vi "Create Group Commands.vi"(7 "VolatusAPI":refnum<class "VolatusAPI.lvclass">, 8 "error in (no error)":errorcluster, 9 "Group Name":string, 10 "Local Node":string, 11 "Cluster":refnum<class "Cluster Config.lvclass">) -> (0 "error out":errorcluster, 2 "Commands":T1)   [LabVIEW 2025, in "VolatusControl.lvlib" / "EStop Module.lvclass"]
uses:
  EStop Module.lvclass
  EStop Module.lvclass/EStop Module.ctl
  VolatusConfig/Channel/Channel Config.lvclass
  C:/dev/volatus/mts-volatus-super/libs/lv-volatus/VolatusConfig/VolatusConfigElement/VolatusConfigElement.lvclass
  C:/dev/volatus/mts-volatus-super/libs/lv-volatus/VolatusConfig/Channel/Channel Config.lvclass
  VolatusConfig/Node/Node Config.lvclass
  C:/dev/volatus/mts-volatus-super/libs/lv-volatus/VolatusConfig/Node/Node Config.lvclass
  VolatusConfig/Cluster/Cluster Config.lvclass
  VolatusConfig/Group/Group Config.lvclass
  VolatusConfig/VolatusConfigElement/VolatusConfigElement.lvclass
  messages/CmdDigital/Data.ctl
  messages/CmdDigital/CmdDigital.lvlib
  Volatus/VolatusAPI/VolatusAPI.lvclass
  lv-cdm/CDM-Config/Config Element/Config Element.lvclass
  Digital Group.ctl
  messages/CmdDigitalMultiple/Data.ctl
  messages/CmdDigitalMultiple/CmdDigitalMultiple.lvlib
  Volatus/MessageQ/MessageQ.lvclass
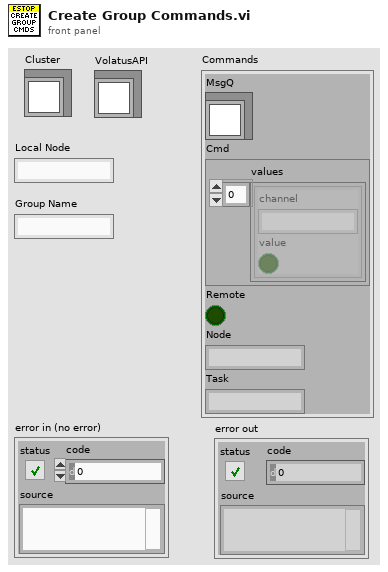
[diagram p1: front panel]
types:
  T1 = typedef "VolatusControl.lvlib/EStop Module.lvclass/Digital Group.ctl" = cluster{"MsgQ":refnum<class "MessageQ.lvclass">, "Cmd":T2, "Remote":bool, "Node":string, "Task":string}
  T2 = typedef "CmdDigitalMultiple.lvlib/Data.ctl" = cluster{"values":T3[]}
  T3 = typedef "CmdDigital.lvlib/Data.ctl" = cluster{"channel":string, "value":bool}
  T4 = typedef "VectoConfig.lvlib/Channel Info.ctl" = cluster{"Name":string, "Group":string, "Owning Node":string, "Owning Task":string, "Resource":string}
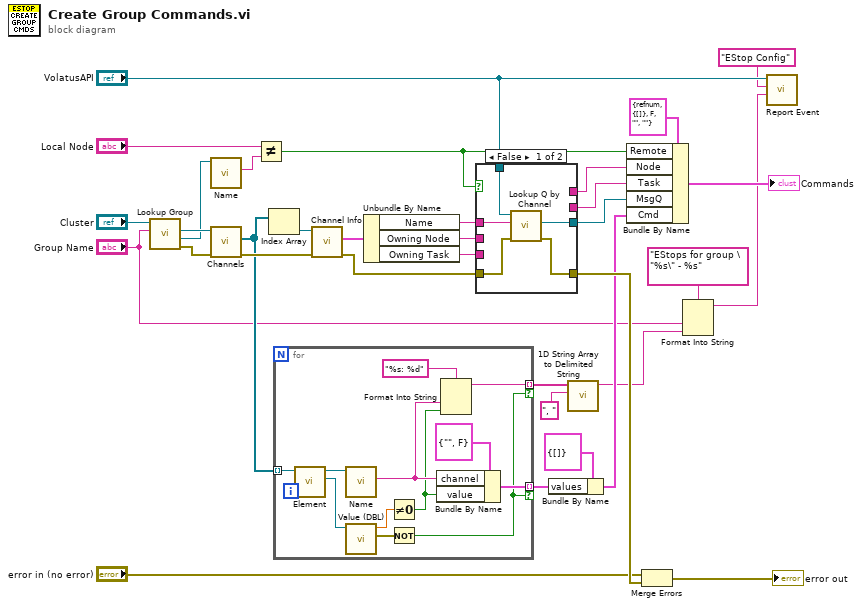
[diagram p0: block diagram]
diagram:
  n1 = call "Lookup Group.vi"("Group Name"="Group Name", "Cluster in"="Cluster") -> ("error out"=w32:errorcluster, "Node"=w29:refnum<class "Node Config.lvclass">, "Group"=w30:refnum<class "Group Config.lvclass">)  [unwired: 6 in, 1 out]
  n2 = call "Name.vi"("VolatusConfigElement in"=w29) -> ("Name"=w26:string)  [unwired: 8 in, 2 out]
  n3 = call "Channels.vi"("error in (no error)"=w32, "Group in"=w30) -> ("error out"=w33:errorcluster, "Channels"=w15:refnum<class "Channel Config.lvclass">[])  [unwired: 7 in, 1 out]
  n4 = Not Equal?(x="Local Node", y=w26) -> (x != y?=w23:bool)
  n5 = Index Array(array=w15) -> (element=w24:refnum<class "Channel Config.lvclass">)  [unwired: 1 in]
  n6 = for {
    tunnel: w15 -> [w46] mode=indexing
    tunnel: [w40] -> w14 mode=indexing if=w35
    tunnel: [w36] -> w8 mode=indexing if=w35
    n7 = call "Element.vi"("VolatusConfigElement in"=w46) -> ("Element"=w45:refnum<class "Config Element.lvclass">, "VolatusConfigElement out"=w44:refnum<class "Channel Config.lvclass">)  [unwired: 9 in]
    n8 = call "Name.vi"("VolatusConfigElement in"=w44) -> ("Name"=w38:string)  [unwired: 8 in, 2 out]
    n9 = call "Value (DBL).vi"("Config Element in"=w45) -> ("error out"=w42:errorcluster, "DBL Value"=w43:dbl)  [unwired: 9 in]
    n10 = Not Equal To 0?(x=w43) -> (x != 0?=w37:bool)
    n11 = Not(x=w42) -> (.not. x?=w35:bool)
    n12 = Bundle By Name(cluster=T3 {"channel"="", "value"=FALSE}, "channel"=w38, "value"=w37) -> (w40:T3)
    n13 = Format Into String(format string="%s: %d", w38, w37) -> (resulting string=w36:string)  [unwired: 2 in, 1 out]
  }
  n14 = call "Channel Info.vi"("error in (no error)"=w33, "Channel in"=w24) -> ("error out"=w9:errorcluster, "Channel Info"=w22:T4)  [unwired: 7 in, 1 out]
  n15 = Unbundle By Name(w22) -> ("Name"=w17:string, "Owning Node"=w20:string, "Owning Task"=w21:string)
  n16 = case shown="False" w23 {
    tunnel: w21 -> [_ w53]
    tunnel: w20 -> [_ w54]
    tunnel: "VolatusAPI" -> [w50 _]
    tunnel: [_ w54] -> w19
    tunnel: [_ w53] -> w18
    tunnel: w17 -> [w51 _]
    tunnel: [w49 _] -> w16
    tunnel: w9 -> [w48 w52]
    tunnel: [w47 w52] -> w34
    frame False {
      n17 = call "Lookup Q by Channel.vi"("error in (no error)"=w48, "Channel Name"=w51, "VolatusAPI in"=w50) -> ("error out"=w47:errorcluster, "MessageQ"=w49:refnum<class "MessageQ.lvclass">)  [unwired: 5 in, 2 out]
    }
    frame True {
    }
  }
  n18 = Bundle By Name(cluster=T2 {"values"=[]} ("Cmd"), "values"=w14) -> (w12:T2)
  n19 = call <vilib>:"1D String Array to Delimited String.vi"("delimiter"=", ", "string array"=w8) -> ("delimited string"=w5:string)  [unwired: 9 in]
  n20 = Bundle By Name(cluster=T1 {"MsgQ"=refnum, "Cmd"={"values"=[]}, "Remote"=FALSE, "Node"="", "Task"=""} ("Commands"), "Remote"=w23, "Node"=w19, "Task"=w18, "MsgQ"=w16, "Cmd"=w12) -> (→"Commands":T1)
  n21 = Merge Errors("error in (no error)", w34) -> (→"error out":errorcluster)
  n22 = Format Into String(format string="EStops for group \"%s\" - %s", "Group Name", w5) -> (resulting string=w2:string)  [unwired: 2 in, 1 out]
  n23 = call "Report Event.vi"("Message"=w2, "Context"="EStop Config", "VolatusAPI in"="VolatusAPI") -> ()  [unwired: 7 in, 2 out]
